vi "TCP Server New.vi"(8 "error in (no error)":errorcluster, 10 "Data in":T1) -> (0 "error out":errorcluster, 3 "TCP Server RefNum":refnum<class "JKI TCP Server.lvclass">)   [LabVIEW 2020, in "JKI TCP Server.lvclass"]
doc: "Initializes the GOOP object"
uses:
  JKI TCP Server.lvclass
  _Data Structures/TCP Server Data.ctl
  _Data Structures/TCP Server Listener Info Cluster.ctl
  _Data Structures/TCP Server Connection Info Cluster.ctl
  _Data Structures/TCP Server Handler RefNum.ctl
panel:
  # "OpenGOOP New.vi\n\nInitializes the GOOP object\n\nCopyright (C) 2002 Jim Kring jim@jimkring.com\n\nPlease visit http://www.OpenG.org to learn about the\nOpen Source LabVIEW software movement.\n\nThis library is free software; you can redistribute it and/or\nmodify it under the terms of the GNU Lesser General Public\nLicense as published by the Free Software Foundation; either\nversion 2.1 of the License, or (at your option) any later version.\nThis library is distributed in the hope that it will be useful,\nbut WITHOUT ANY WARRANTY; without even the implied warranty of\nMERCHANTABILITY or FITNESS FOR A PARTICULAR PURPOSE. See the GNU\nLesser General Public License for more details.\nYou should have received a copy of the GNU Lesser General Public\nLicense along with this library; if not, write to the Free Software\nFoundation, Inc., 59 Temple Place, Suite 330, Boston, MA 02111-1307 USA"
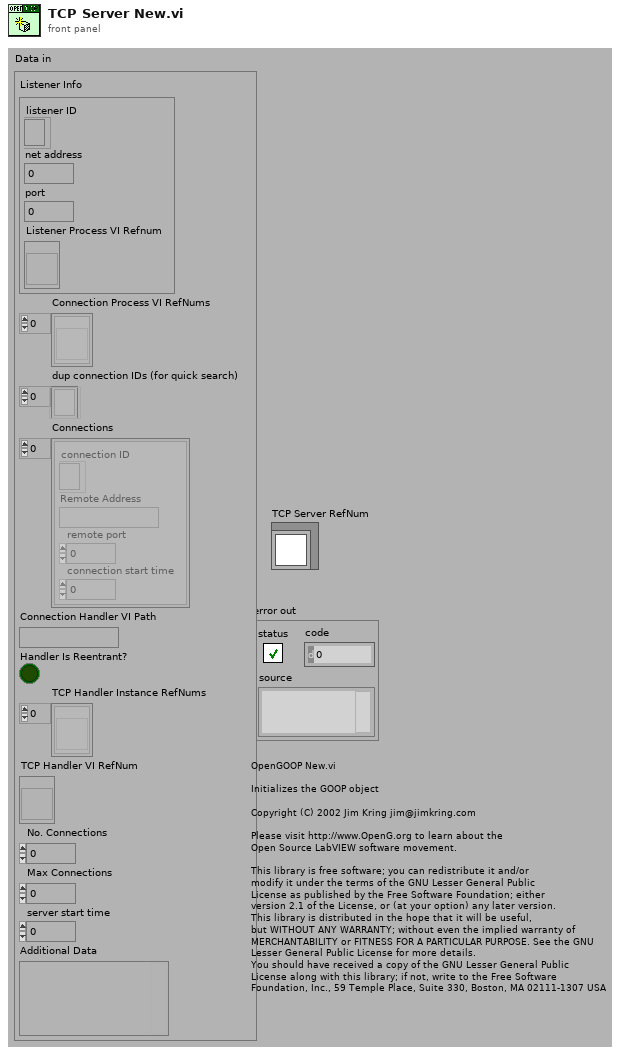
[diagram p1: front panel]
types:
  T1 = typedef "JKI TCP Server.lvclass/TCP Server Data.ctl" = cluster{"Listener Info":T2, "Connection Process VI RefNums":refnum<vi>[], "dup connection IDs (for quick search)":refnum<k5>[], "Connections":T3[], "Connection Handler VI Path":path, "Handler Is Reentrant?":bool, "TCP Handler Instance RefNums":T4[], "TCP Handler VI RefNum":T4, "No. Connections":u32, "Max Connections":u32, "server start time":u32, "Additional Data":variant}
  T2 = typedef "JKI TCP Server.lvclass/TCP Server Listener Info Cluster.ctl" = cluster{"listener ID":refnum<k5>, "net address":u32, "port":u16, "Listener Process VI Refnum":refnum<vi>}
  T3 = typedef "JKI TCP Server.lvclass/TCP Server Connection Info Cluster.ctl" = cluster{"connection ID":refnum<k5>, "Remote Address":string, "remote port":u16, "connection start time":u32}
  T4 = typedef "JKI TCP Server.lvclass/TCP Server Handler RefNum.ctl" = refnum<vi>
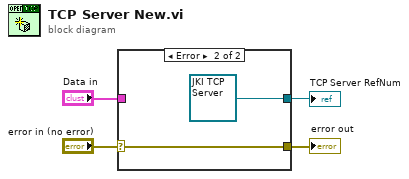
[diagram p0: block diagram]
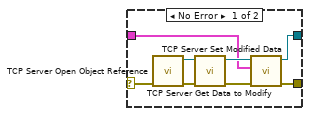
[diagram p2: hidden frame]
diagram:
  n1 = case shown="Error" "error in (no error)" {
    selector: "error in (no error)" -> [w5 w14]
    tunnel: [w11 w14] -> w4
    tunnel: "Data in" -> [w8 _]
    tunnel: [w10 refnum<class "JKI TCP Server.lvclass"> refnum ("TCP Server RefNum")] -> w1
    frame No Error {
      n2 = call "TCP Server Open Object Reference.vi"("error in (no error)"=w5) -> ("error out"=w7:errorcluster, "TCP Server Refnum"=w6:refnum<class "JKI TCP Server.lvclass">)  [unwired: 9 in]
      n3 = call "TCP Server Get Data to Modify.vi"("error in (no error)"=w7, "RefNum"=w6) -> ("error out"=w12:errorcluster, "dup RefNum"=w9:refnum<class "JKI TCP Server.lvclass">)  [unwired: 6 in, 2 out]
      n4 = call "TCP Server Set Modified Data.vi"("error in (no error)"=w12, "Data in"=w8, "RefNum"=w9) -> ("error out"=w11:errorcluster, "dup RefNum"=w10:refnum<class "JKI TCP Server.lvclass">)  [unwired: 7 in]
    }
    frame Error {
    }
  }
  "error out" <- w4
  "TCP Server RefNum" <- w1
